vi "appendText.vi"(8 "error in (no error)":errorcluster, 9 "Style":refnum<class "Style.lvclass">, 10 "Text":string, 11 "MS-Word in":refnum<class "MS-Word.lvclass">) -> (0 "error out":errorcluster, 3 "MS-Word out":refnum<class "MS-Word.lvclass">)   [LabVIEW 2017, in "LabVIEW NPOI.lvlib" / "MS-Word.lvclass"]
uses:
  MS-Word.lvclass
  Styles/Style/Style.lvclass
  MS-Word.lvclass/MS-Word.ctl
  xwpfDocument/xwpfDocument.lvclass
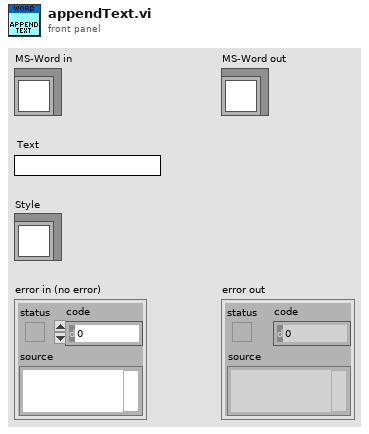
[diagram p1: front panel]
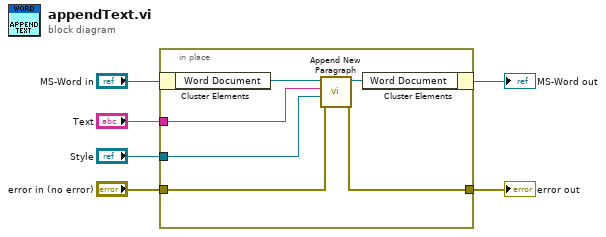
[diagram p0: block diagram]
diagram:
  n1 = in-place {
    in-place-border: "error in (no error)" -> [w10]
    in-place-border: [w9] -> w3
    in-place-border: "Text" -> [w8]
    in-place-border: "Style" -> [w7]
    n2 = in-place-cluster #1("MS-Word in") -> ("Word Document"=w12:refnum<class "xwpfDocument.lvclass">)
    n3 = call "Append New Paragraph.vi"("error in (no error)"=w10, "Paragraph.Style"=w7, "Paragraph.Text"=w8, "xwpfDocument in"=w12) -> ("error out"=w9:errorcluster, "xwpfDocument out"=w11:refnum<class "xwpfDocument.lvclass">)  [unwired: 6 in]
    n4 = in-place-cluster #1("Word Document"=w11) -> (→"MS-Word out":refnum<class "MS-Word.lvclass">)
  }
  "error out" <- w3
